vi "Arduino Reader.vi"() -> ()   [LabVIEW 2013]
uses:
  <vilib>/Instr/_visa.llb/VISA Configure Serial Port (Instr).vi
  <vilib>/ptbypt/NI_PtbyPt.lvlib
panel:
  in  "Item 3":string="FILZ"
  in  "Item 2":string="FILY"
  in  "Item":string="FILX"
  out "Z":dbl(graph)
  out "Y":dbl(graph)
  out "X":dbl(graph)
  in  "sample length":i32=10
  out "Waveform Chart":T1(graph)
  out "Raw":string
  in  "baud rate (9600)":u32=9600
  in  "VISA resource name":refnum<visa-resource-name>
  in  "Stop Button":bool
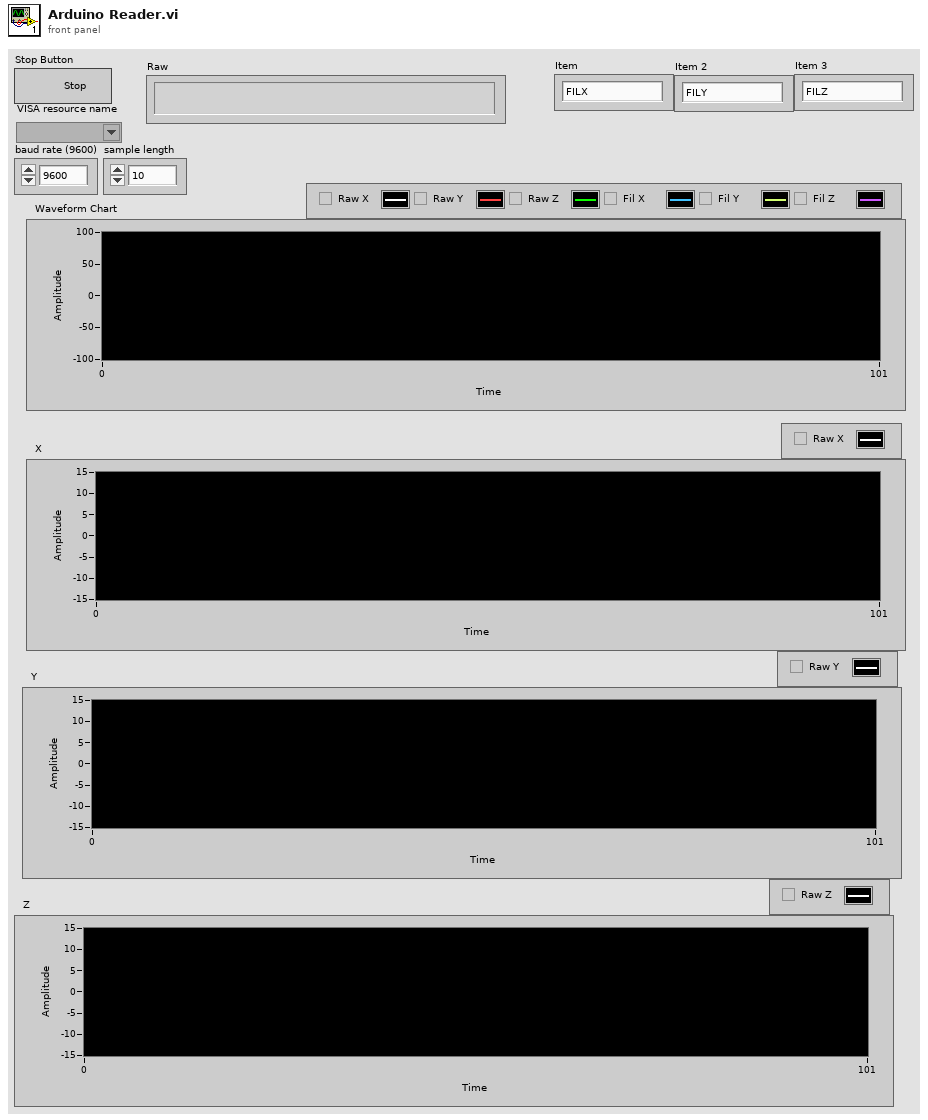
[diagram p1: front panel]
types:
  T1 = cluster{"Value":dbl, "Value":dbl, "Value":dbl, "mean":dbl, "mean":dbl, "mean":dbl}
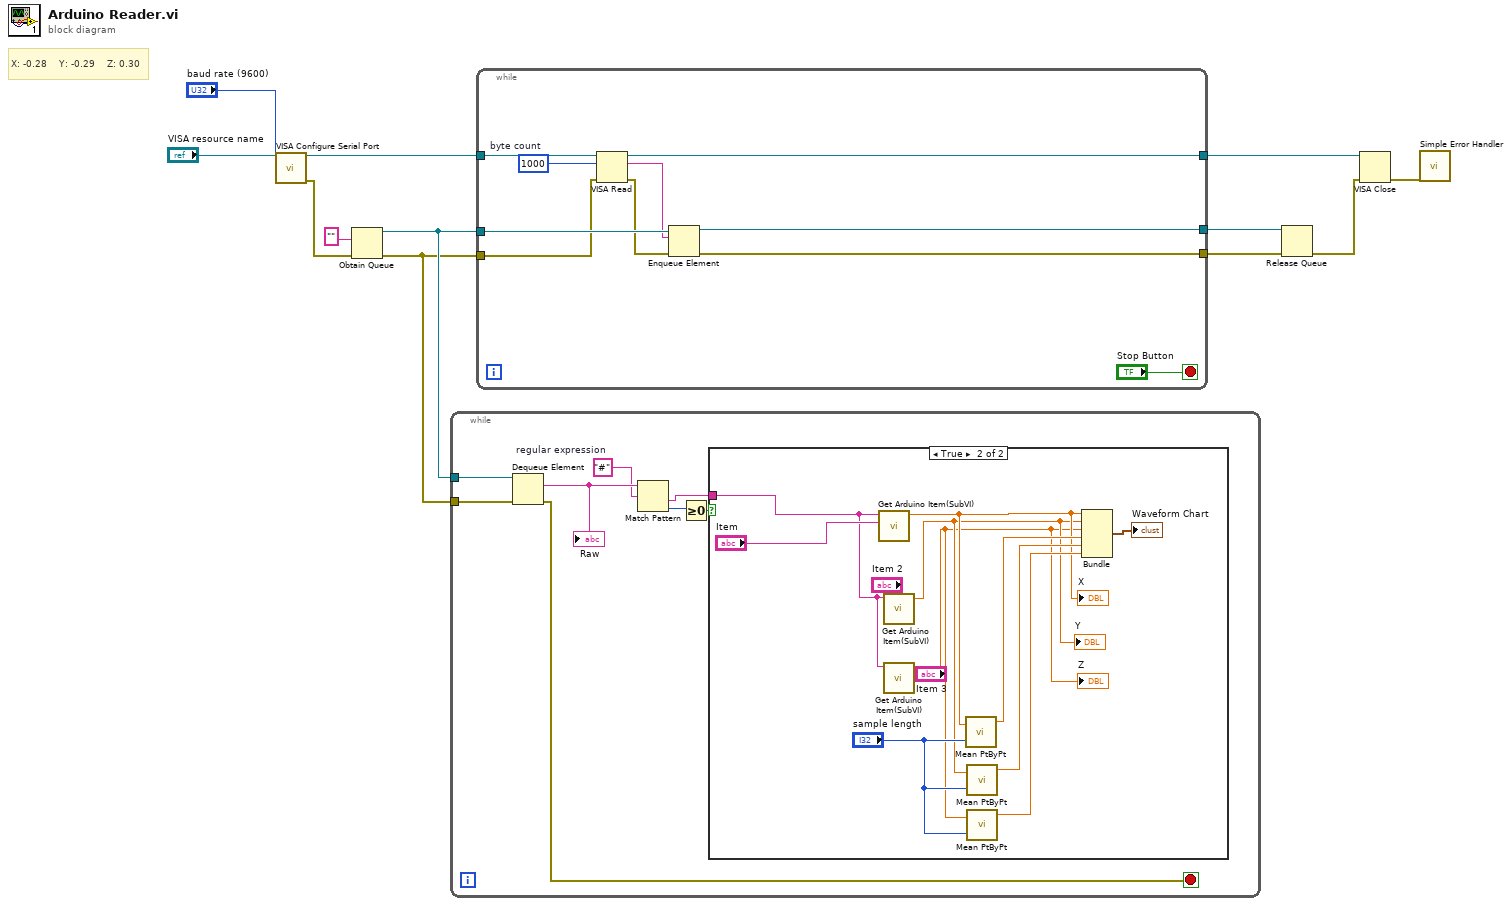
[diagram p0: block diagram]
diagram:
  # "X: -0.28    Y: -0.29    Z: 0.30"
  n1 = call-poly "VISA Configure Serial Port"("VISA resource name"="VISA resource name", "baud rate (9600)"="baud rate (9600)") -> ("VISA resource name out"=w7:refnum<visa-resource-name>, "error out"=w9:errorcluster)  [unwired: 12 in]
  n2 = Obtain Queue(element data type="", error in (no error)=w9) -> (queue out=w2:refnum<queue>, error out=w1:errorcluster)  [unwired: 3 in, 1 out]
  n3 = while {
    tunnel: w2 -> [w19]
    tunnel: w1 -> [w18]
    stop <- w20 stop-if-true
    w16 = "#"  # regular expression
    n4 = Dequeue Element(queue=w19, error in (no error)=w18) -> (element=w17:string, error out=w20:errorcluster)  [unwired: 1 in, 2 out]
    "Raw" <- w17
    n5 = Match Pattern(string=w17, regular expression=w16) -> (after substring=w13:string, offset past match=w15:i32)  [unwired: 1 in, 2 out]
    n6 = Greater Or Equal To 0?(x=w15) -> (x >= 0?=w14:bool)
    n7 = case shown="True" w14 {
      tunnel: w13 -> [_ w29]
      frame False {
      }
      frame True {
        n8 = call "Get Arduino Item(SubVI).vi"("Item"="Item", "String"=w29) -> ("Value"=w23:dbl)  [unwired: 9 in]
        "X" <- w23
        n9 = call "Get Arduino Item(SubVI).vi"("Item"="Item 2", "String"=w29) -> ("Value"=w22:dbl)  [unwired: 9 in]
        "Y" <- w22
        n10 = call "Get Arduino Item(SubVI).vi"("Item"="Item 3", "String"=w29) -> ("Value"=w21:dbl)  [unwired: 9 in]
        "Z" <- w21
        n11 = call <vilib>:"Mean PtByPt.vi"("x"=w23, "sample length"="sample length") -> ("mean"=w27:dbl)  [unwired: 2 in, 1 out]
        n12 = call <vilib>:"Mean PtByPt.vi"("x"=w22, "sample length"="sample length") -> ("mean"=w26:dbl)  [unwired: 2 in, 1 out]
        n13 = call <vilib>:"Mean PtByPt.vi"("x"=w21, "sample length"="sample length") -> ("mean"=w25:dbl)  [unwired: 2 in, 1 out]
        n14 = Bundle("Value"=w23, "Value"=w22, "Value"=w21, "mean"=w27, "mean"=w26, "mean"=w25) -> (→"Waveform Chart":T1)  [unwired: 1 in]
      }
    }
  }
  n15 = while {
    tunnel: w2 -> [w41]
    tunnel: [w40] -> w12
    tunnel: w1 -> [w38]
    tunnel: w7 -> [w39]
    tunnel: [w34] -> w6
    tunnel: [w33] -> w5
    stop <- "Stop Button" stop-if-true
    w35 = u32 1000  # byte count
    n16 = VISA Read(VISA resource name=w39, byte count=w35, error in (no error)=w38) -> (VISA resource name out=w33:refnum<visa-resource-name>, read buffer=w36:string, error out=w37:errorcluster)  [unwired: 1 out]
    n17 = Enqueue Element(queue=w41, element=w36, error in (no error)=w37) -> (queue out=w40:refnum<queue>, error out=w34:errorcluster)  [unwired: 1 in, 1 out]
  }
  n18 = Release Queue(queue=w12, error in (no error)=w6) -> (error out=w4:errorcluster)  [unwired: 1 in, 2 out]
  n19 = VISA Close(VISA resource name=w5, error in (no error)=w4) -> (error out=w3:errorcluster)
  n20 = call <vilib>:"Simple Error Handler.vi"("error in (no error)"=w3) -> ()  [unwired: 4 in, 5 out]
